vi "Pre-Build Action.vi"(6 "Top Level/Always Included VIs":path[](array[path]), 7 "Main Destination Path":path, 9 "Target Name":string, 10 "Build Specification Name":string, 11 "Project Path":path=path "C:/LabVIEW Code/TALOS/talos/TALOS.lvproj") -> (0 "error out":errorcluster)   [LabVIEW 2020]
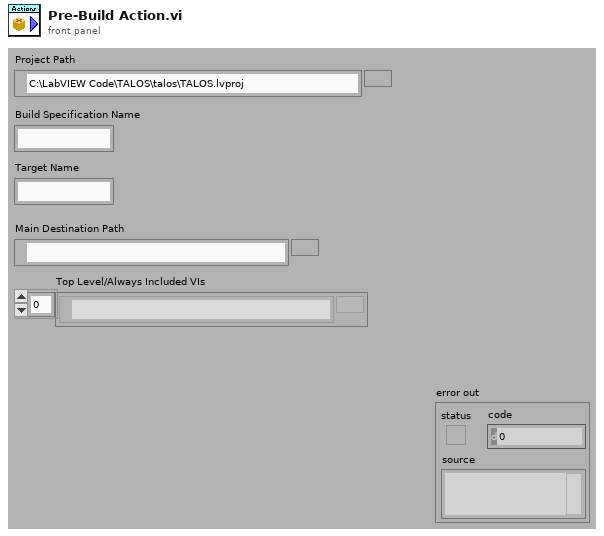
[diagram p1: front panel]
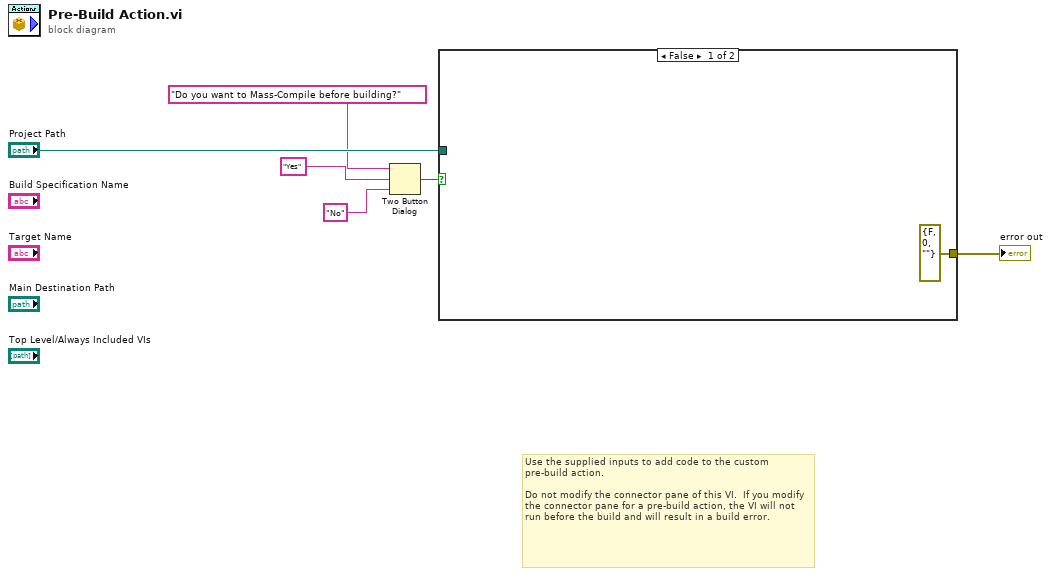
[diagram p0: block diagram]
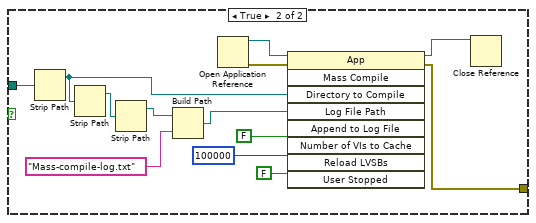
[diagram p2: hidden frame]
diagram:
  # "Use the supplied inputs to add code to the custom pre-build action.\n\nDo not modify the connector pane of this VI.  If you modify the connector pane for a pre-build action, the VI will not run before the build and will result in a build error."
  n1 = Two Button Dialog(message="Do you want to Mass-Compile before building?", 1:"No" ("F button name (\"Cancel\")"), 2:"Yes" ("T button name (\"OK\")")) -> (T button?=w4:bool)
  n2 = case shown="False" w4 {
    tunnel: "Project Path" -> [_ w18]
    tunnel: [errorcluster {"status"=FALSE, "code"=0, "source"=""} ("error out") w12] -> w5
    frame False {
    }
    frame True {
      n3 = Strip Path(path=w18) -> (stripped path=w15:path)  [unwired: 1 out]
      n4 = Strip Path(path=w15) -> (stripped path=w9:path)  [unwired: 1 out]
      n5 = Strip Path(path=w9) -> (stripped path=w8:path)  [unwired: 1 out]
      n6 = Build Path(base path=w8, name or relative path="Mass-compile-log.txt") -> (appended path=w13:path)
      n7 = Open Application Reference() -> (0:w19:errorcluster, 3:w20:refnum<vi>)  [unwired: 4 in]
      n8 = invoke class="App" method="Mass Compile"(reference=w20, error in=w19, "Directory to Compile"=w15, "Log File Path"=w13, "Append to Log File"=FALSE, "Number of VIs to Cache"=u32 100000, "Reload LVSBs"=FALSE) -> (reference out=w11:refnum<vi>, error out=w12:errorcluster)  [unwired: 2 in, 7 out]
      n9 = Close Reference(reference=w11) -> ()  [unwired: 1 in, 1 out]
    }
  }
  "error out" <- w5
